vi "VIH - CHM Project - HHP Support - Set Key.vi"(6 "key/value separator (T)":bool=TRUE, 7 "Section":string, 8 "error in":errorcluster, 9 "Value":string, 10 "Key":string, 11 "queue":T1) -> (0 "error out":errorcluster, 3 "dup queue":T1)   [LabVIEW 2014]
doc: "::: VI Helpeks :::\nCopyright (c) 2000-2026 Konstantin Shifershteyn. All rights reserved."
uses:
  VIH - CHM Project - HHP Support - Queue Refnum.ctl
  VIH - CHM Project - HHP Support - Config Data Cluster.ctl
panel:
  # "VI Helpeks\nCopyright (c) 2012-2026 Konstantin Shifershteyn"
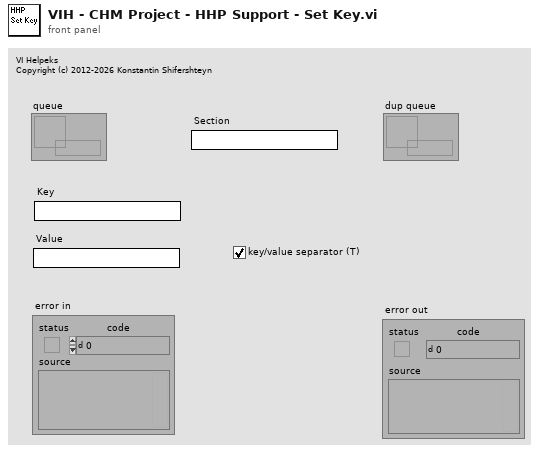
[diagram p1: front panel]
types:
  T1 = typedef "VIH - CHM Project - HHP Support - Queue Refnum.ctl" = refnum<queue>
  T2 = typedef "VIH - CHM Project - HHP Support - Config Data Cluster.ctl" = cluster{"Fille path":path, "sections":cluster{"Sec name":string, "key-values":string[][]}[]}
  T3 = cluster{"Sec name":string, "key-values":string[][]}[]
  T4 = cluster{"Sec name":string, "key-values":string[][]}
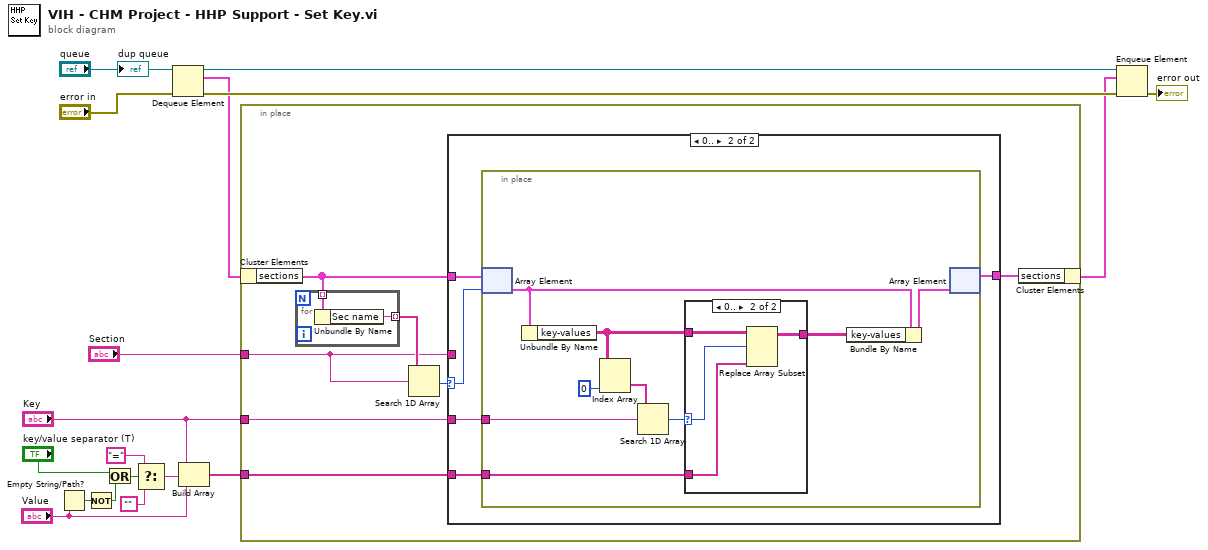
[diagram p0: block diagram]
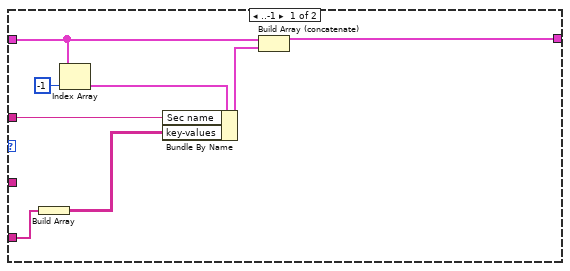
[diagram p2: hidden frame]
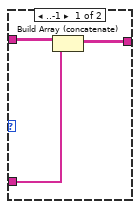
[diagram p3: hidden frame]
diagram:
  n1 = Empty String/Path?(string/path="Value") -> (empty?=w10:bool)
  n2 = Not(x=w10) -> (.not. x?=w9:bool)
  n3 = Or(x="key/value separator (T)", y=w9) -> (x .or. y?=w7:bool)
  n4 = Select(t="=", s=w7, f="") -> (s? t:f=w3:string)
  n5 = Dequeue Element(queue="queue", error in (no error)="error in") -> (queue out=w18:T1, element=w13:T2, error out=w15:errorcluster)  [unwired: 1 in, 1 out]
  n6 = Build Array("Key", w3, "Value") -> (w2:string[])
  n7 = in-place {
    in-place-border: "Section" -> [w21]
    in-place-border: w2 -> [w20]
    in-place-border: "Key" -> [w19]
    n8 = in-place-cluster #1(w13) -> ("sections"=w23:T3)
    n9 = for {
      tunnel: w23 -> [w56] mode=indexing
      tunnel: [w55] -> w25 mode=indexing
      n10 = Unbundle By Name(w56) -> ("Sec name"=w55:string)
    }
    n11 = Search 1D Array(1D array=w25, element=w21) -> (index of element=w24:i32)  [unwired: 1 in]
    n12 = case shown="0.." w24 {
      selector: w24 -> [_ w36]
      tunnel: w23 -> [w33 w37]
      tunnel: [w29 w35] -> w22
      tunnel: w21 -> [w28 _]
      tunnel: w20 -> [w27 w34]
      tunnel: w19 -> [_ w38]
      frame ..-1 {
        n13 = Build Array(w27) -> (w26:string[][])
        n14 = Index Array(array=w33, index=-1) -> (element=w31:T4)
        n15 = Bundle By Name(cluster=w31, "Sec name"=w28, "key-values"=w26) -> (w30:T4)
        n16 = Build Array (concatenate)(w33, w30) -> (w29:T3)
      }
      frame 0.. {
        n17 = in-place {
          in-place-border: w38 -> [w46]
          in-place-border: w34 -> [w40]
          n18 = in-place-array #2(w37, w36) -> (w43:T4)
          n19 = Unbundle By Name(w43) -> ("key-values"=w41:string[][])
          n20 = Index Array(array=w41, index (col)=0 ("disabled index (col)")) -> (element=w45:string[])  [unwired: 1 in]
          n21 = Search 1D Array(1D array=w45, element=w46) -> (index of element=w44:i32)  [unwired: 1 in]
          n22 = case shown="0.." w44 {
            selector: w44 -> [_ w53]
            tunnel: w41 -> [w50 w54]
            tunnel: w40 -> [w49 w52]
            tunnel: [w48 w51] -> w39
            frame ..-1 {
              n23 = Build Array (concatenate)(w50, w49) -> (w48:string[][])
            }
            frame 0.. {
              n24 = Replace Array Subset(array=w54, new element=w52, index (row)=w53) -> (w51:string[][])  [unwired: 1 in]
            }
          }
          n25 = Bundle By Name(cluster=w43, "key-values"=w39) -> (w42:T4)
          n26 = in-place-array #2(w42) -> (w35:T3)  [unwired: 1 out]
        }
      }
    }
    n27 = in-place-cluster #1("sections"=w22) -> (w12:T2)
  }
  n28 = Enqueue Element(queue=w18, element=w12, error in (no error)=w15) -> (error out=→"error out":errorcluster)  [unwired: 1 in, 2 out]
  "dup queue" <- "queue"
